vi "DestroySelfReference.vi"(8 "error in (no error)":errorcluster, 11 "Microscope":refnum<class "Microscope.lvclass">) -> (0 "error out":errorcluster, 3 "Microscope out":refnum<class "Microscope.lvclass">)   [LabVIEW 2013, in "Microscope.lvclass"]
doc: "JKI State Machine Objects (SMO) 1.0.0.5\nJKI - JKI\nCopyright (c) 2016, JKI"
uses:
  Microscope.lvclass
  <vilib>/JKI/JKI SMO/SMO/SMO.lvclass
panel:
  # "For instructions on how to use the JKI State Machine Objects, examples and video tutorials, visit:\nhttp://jki.net/state-machine-objects/\n\nJKI State Machine Objects™\nhttp://jki.net/state-machine-objects/\nCopyright (C) 2005-2015, JKI <info@jki.net>\nALL RIGHTS RESERVED"
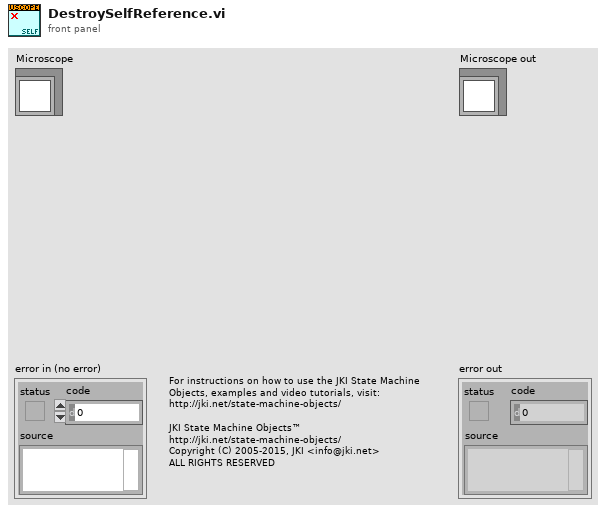
[diagram p1: front panel]
types:
  T1 = typedef "Microscope.lvclass/PrivateData--Ref.ctl" = refnum<data-value>
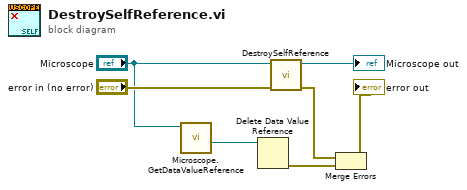
[diagram p0: block diagram]
diagram:
  n1 = call "Microscope.GetDataValueReference.vi"("Microscope"="Microscope") -> ("Ref"=w1:T1)  [unwired: 10 in]
  n2 = Delete Data Value Reference(data value reference=w1) -> (error out=w4:errorcluster)  [unwired: 1 in, 1 out]
  n3 = call-parent "DestroySelfReference.vi"("error in (no error)"="error in (no error)", "SMO"="Microscope") -> ("error out"=w3:errorcluster, "SMO out"=→"Microscope out":refnum<class "Microscope.lvclass">)  [unwired: 8 in]
  n4 = Merge Errors(w3, w4) -> (→"error out":errorcluster)
